vi "Enable T1.vi"(8 "error in (no error)":errorcluster caption="错误输入（无错误）", 9 "uMask16":u16, 10 "nBoard":i32, 11 "nDevId":i32) -> (0 "error out":errorcluster caption="错误输出", 3 "function return":i32)   [LabVIEW 2017, in "smncsftmt.lvlib"]
doc: "__declspec(dllexport) int EnableT1(int nDevId, int nBoard, unsigned short uMask16);"
uses:
  smncsftmt.lvlib
  smncsftmt.dll
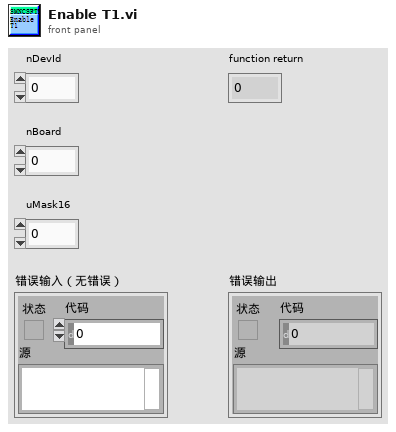
[diagram p1: front panel]
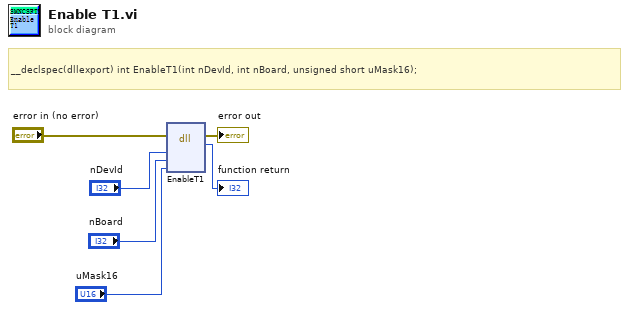
[diagram p0: block diagram]
diagram:
  # "__declspec(dllexport) int EnableT1(int nDevId, int nBoard, unsigned short uMask16);"
  n1 = dll-call lib="PTH2oabs CUsersaDesktop\nLABVIEW范例National InstrumentsLabVIEW 2017user.lib\tsmncsftmtsmncsftmt.*" fn="EnableT1"(error in="error in (no error)", "nDevId"="nDevId", "nBoard"="nBoard", "uMask16"="uMask16") -> (error out=→"error out":errorcluster, "返回类型"=→"function return":i32)  [unwired: 5 in, 1 out]
